vi "close_service.vi"(8 "error in (no error)":errorcluster, 11 "system.logging (in)":refnum<class "system.logging.lvclass">) -> (0 "error out":errorcluster, 3 "system.logging (out)":refnum<class "system.logging.lvclass">)   [LabVIEW 2021, in "system.logging.lvclass"]
uses:
  system.logging.lvclass
  log_stream.ctl
  service_commands.ctl
  log_entry.ctl
  severity.ctl
  system.logging.lvclass/system.logging.ctl
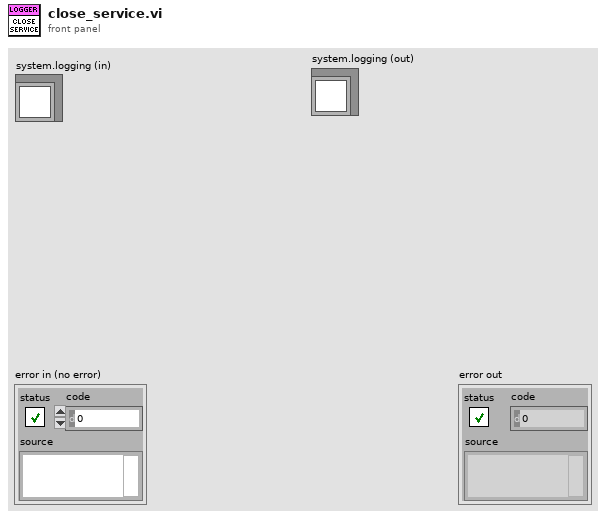
[diagram p1: front panel]
types:
  T1 = typedef "system.logging.lvclass/severity.ctl" = enum8{"trace", "debug", "info", "warning", "error"}
  T2 = typedef "system.logging.lvclass/service_commands.ctl" = enum16{"close", "log"}
  T3 = typedef "system.logging.lvclass/log_stream.ctl" = cluster{"command":T2, "log_entry":T4}
  T4 = typedef "system.logging.lvclass/log_entry.ctl" = cluster{"severity":T1, "message":string, "origin":string, "datetime":timestamp}
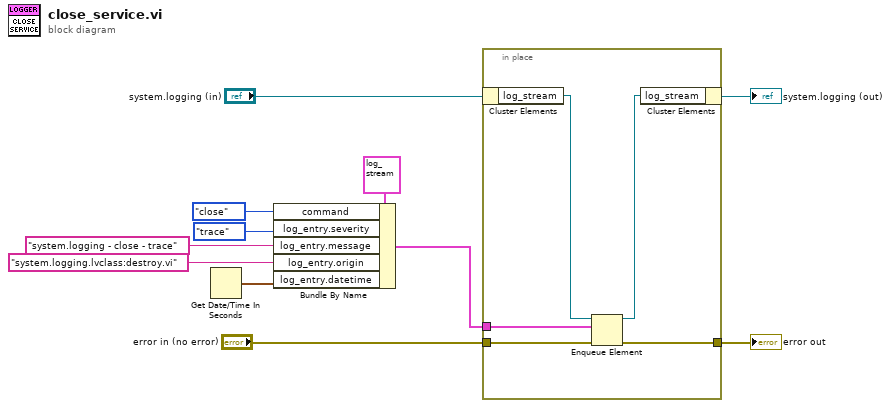
[diagram p0: block diagram]
diagram:
  n1 = Get Date/Time In Seconds() -> (seconds since 1Jan1904=w7:timestamp)
  n2 = Bundle By Name(cluster=T3 {"command"=enum."close", "log_entry"={"severity"=enum."trace", "message"="", "origin"="", "datetime"=timestamp(0 s since 1904-01-01)}} ("element"), "command"=service_commands."close", "log_entry.severity"=severity."trace", "log_entry.message"="system.logging - close - trace", "log_entry.origin"="system.logging.lvclass:destroy.vi", "log_entry.datetime"=w7) -> (w3:T3)
  n3 = in-place {
    in-place-border: "error in (no error)" -> [w16]
    in-place-border: [w15] -> w10
    in-place-border: w3 -> [w14]
    n4 = in-place-cluster #1("system.logging (in)") -> ("log_stream"=w13:refnum<queue>)
    n5 = Enqueue Element(queue=w13, element=w14, error in (no error)=w16) -> (queue out=w12:refnum<queue>, error out=w15:errorcluster)  [unwired: 1 in, 1 out]
    n6 = in-place-cluster #1("log_stream"=w12) -> (→"system.logging (out)":refnum<class "system.logging.lvclass">)
  }
  "error out" <- w10
